vi "close_ref.vi"() -> ()   [LabVIEW 2022 SP3]
panel:
  out "error out":errorcluster
  in  "reference":refnum<vi>
  in  "error in (no error)":errorcluster
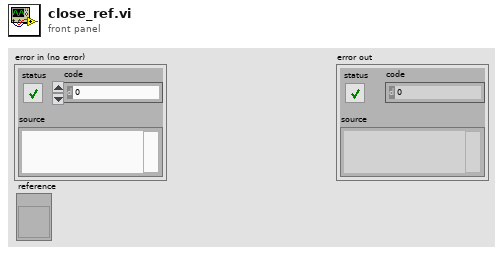
[diagram p1: front panel]
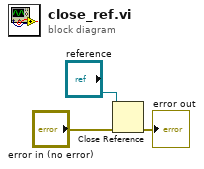
[diagram p0: block diagram]
diagram:
  n1 = Close Reference(reference="reference", error in (no error)="error in (no error)") -> (error out=→"error out":errorcluster)
